vi "loadcell.vi"() -> ()   [LabVIEW 2020]
uses:
  <vilib>/DAQmx/read.llb/DAQmx Read (Analog 1D Wfm NChan NSamp).vi
  <vilib>/DAQmx/miscellaneous.llb/DAQmx Fill In Error Info.vi
panel:
  out "data 3":waveform(dbl)[](graph) caption="data"
  out "channel name(s) out":string[](array[string])
  in  "file path":path
  in  "stop":bool
  in  "data 2":waveform(dbl)[](array[waveform])
  out "data":waveform(dbl)[](graph)
  out "error out 2":errorcluster
  in  "error in (no error)":errorcluster
  out "Tare log":bool
  out "Start log":bool
  out "reconnect":bool
  out "Show message":bool
  in  "Message":string
  in  "No of Samples":dbl
  out "save Path":path
  in  "Tare":bool
  in  "Report":bool
  in  "Refresh Button":bool
  in  "Start Log":bool
  out "No of Sample":dbl
  out "Count":dbl
  out "Samples":dbl
  in  "Machine Load 3":dbl
  in  "Sample Delay":dbl
  in  "Machine Load 2":dbl
  in  "Sample Rate":dbl
  out "Part No":dbl
  out "Total Load":dbl
  out "KG 4":dbl
  out "KG 3":dbl
  out "KG 2":dbl
  out "KG":dbl
  out "Loadcell 4":bool
  out "Loadcell 3":bool
  out "Loadcell 2":bool
  out "Loadcell1":bool
  out "Loadcell 4":waveform(dbl)(graph)
  out "Loadcell 3":waveform(dbl)(graph)
  out "Loadcell 2":waveform(dbl)(graph)
  out "Loadcell1":waveform(dbl)(graph)
  # "KG"
  # "MS"
  # "Hz"
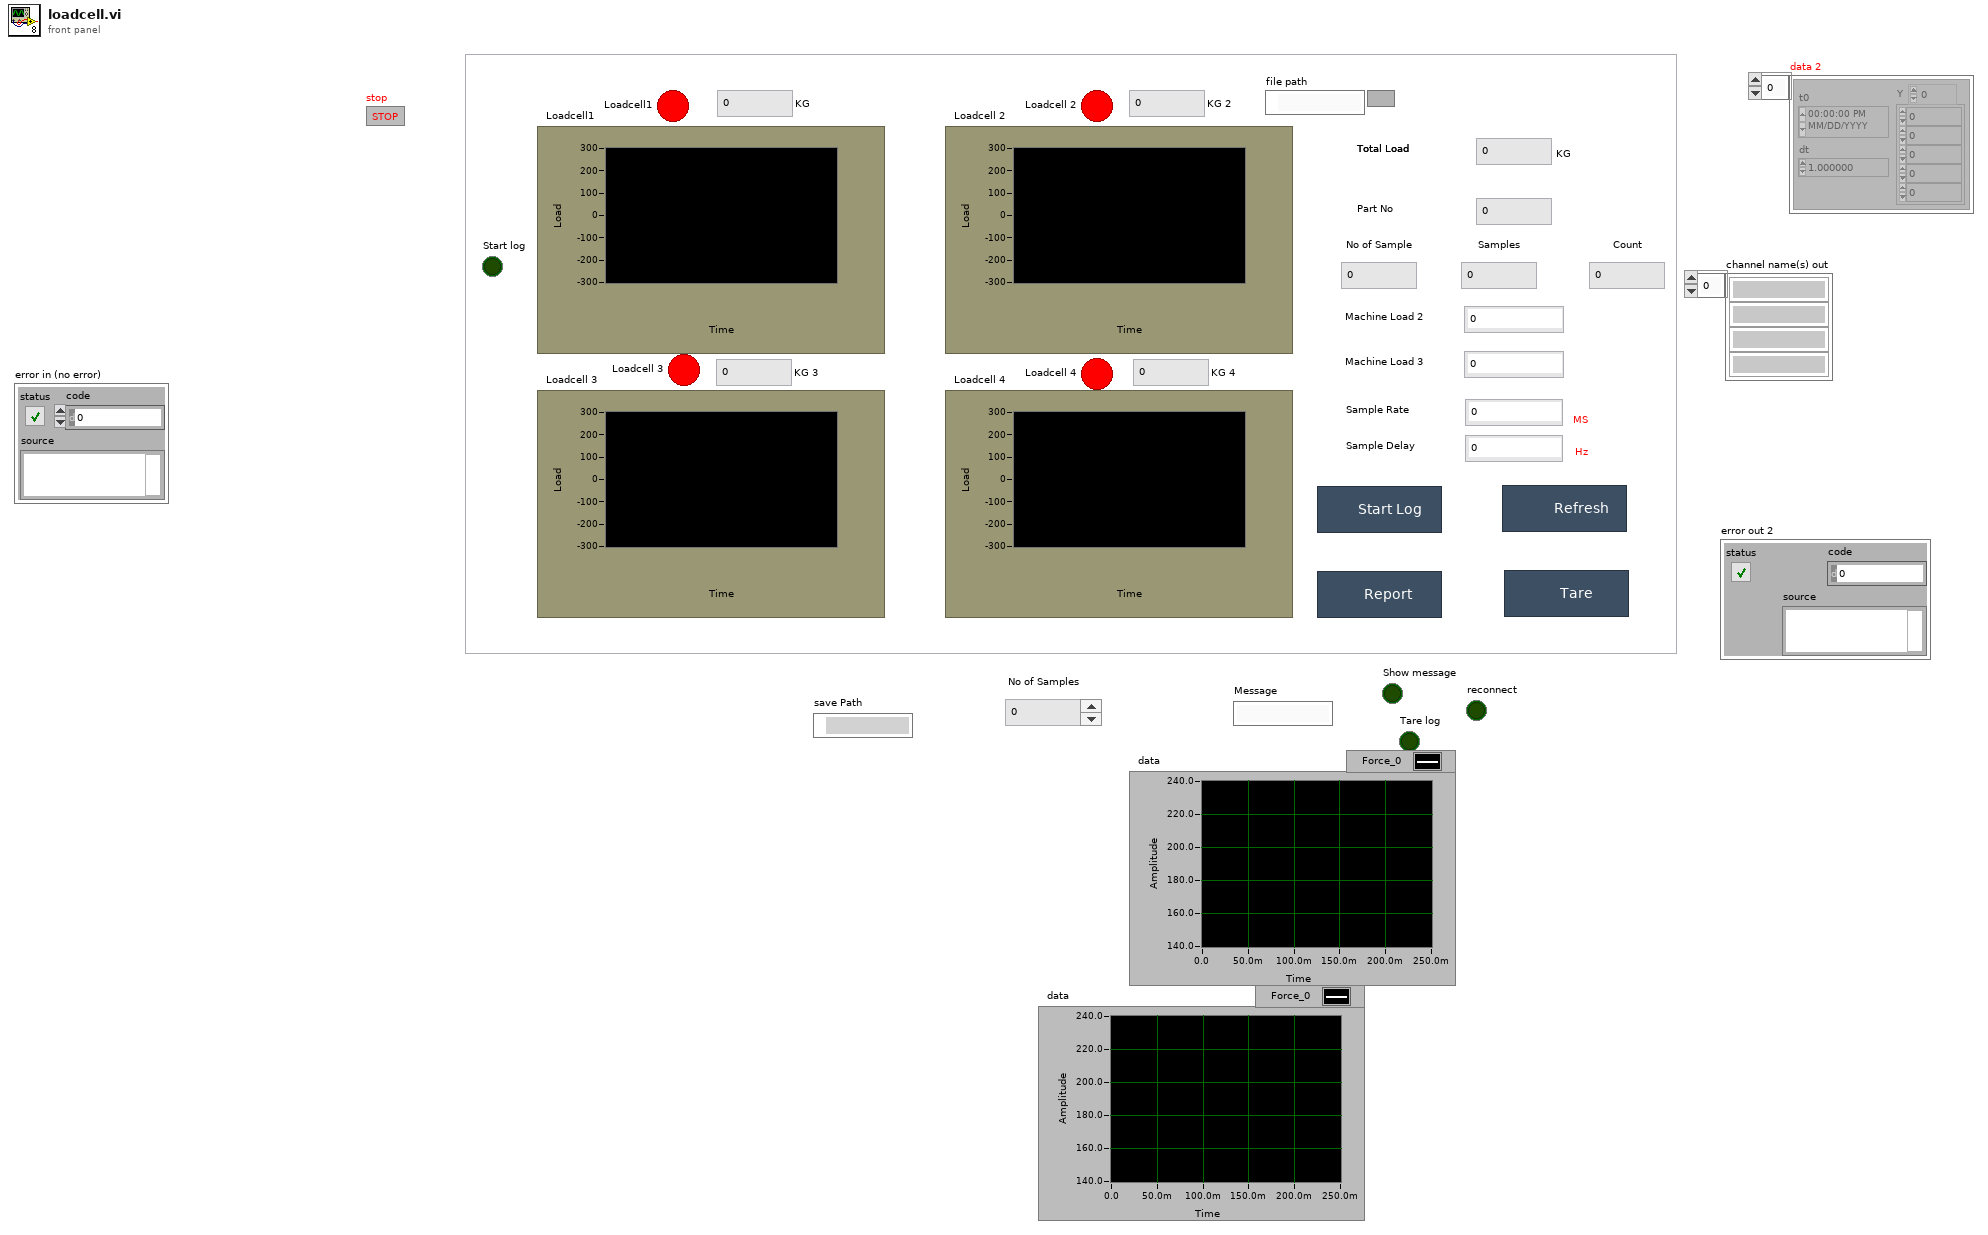
[diagram p1: front panel]
types:
  T1 = enum16{"big-endian, network order", "native, host order", "little-endian"}
  T2 = enum16{"open", "open or create", "create or replace", "create", "open (read-only)"}
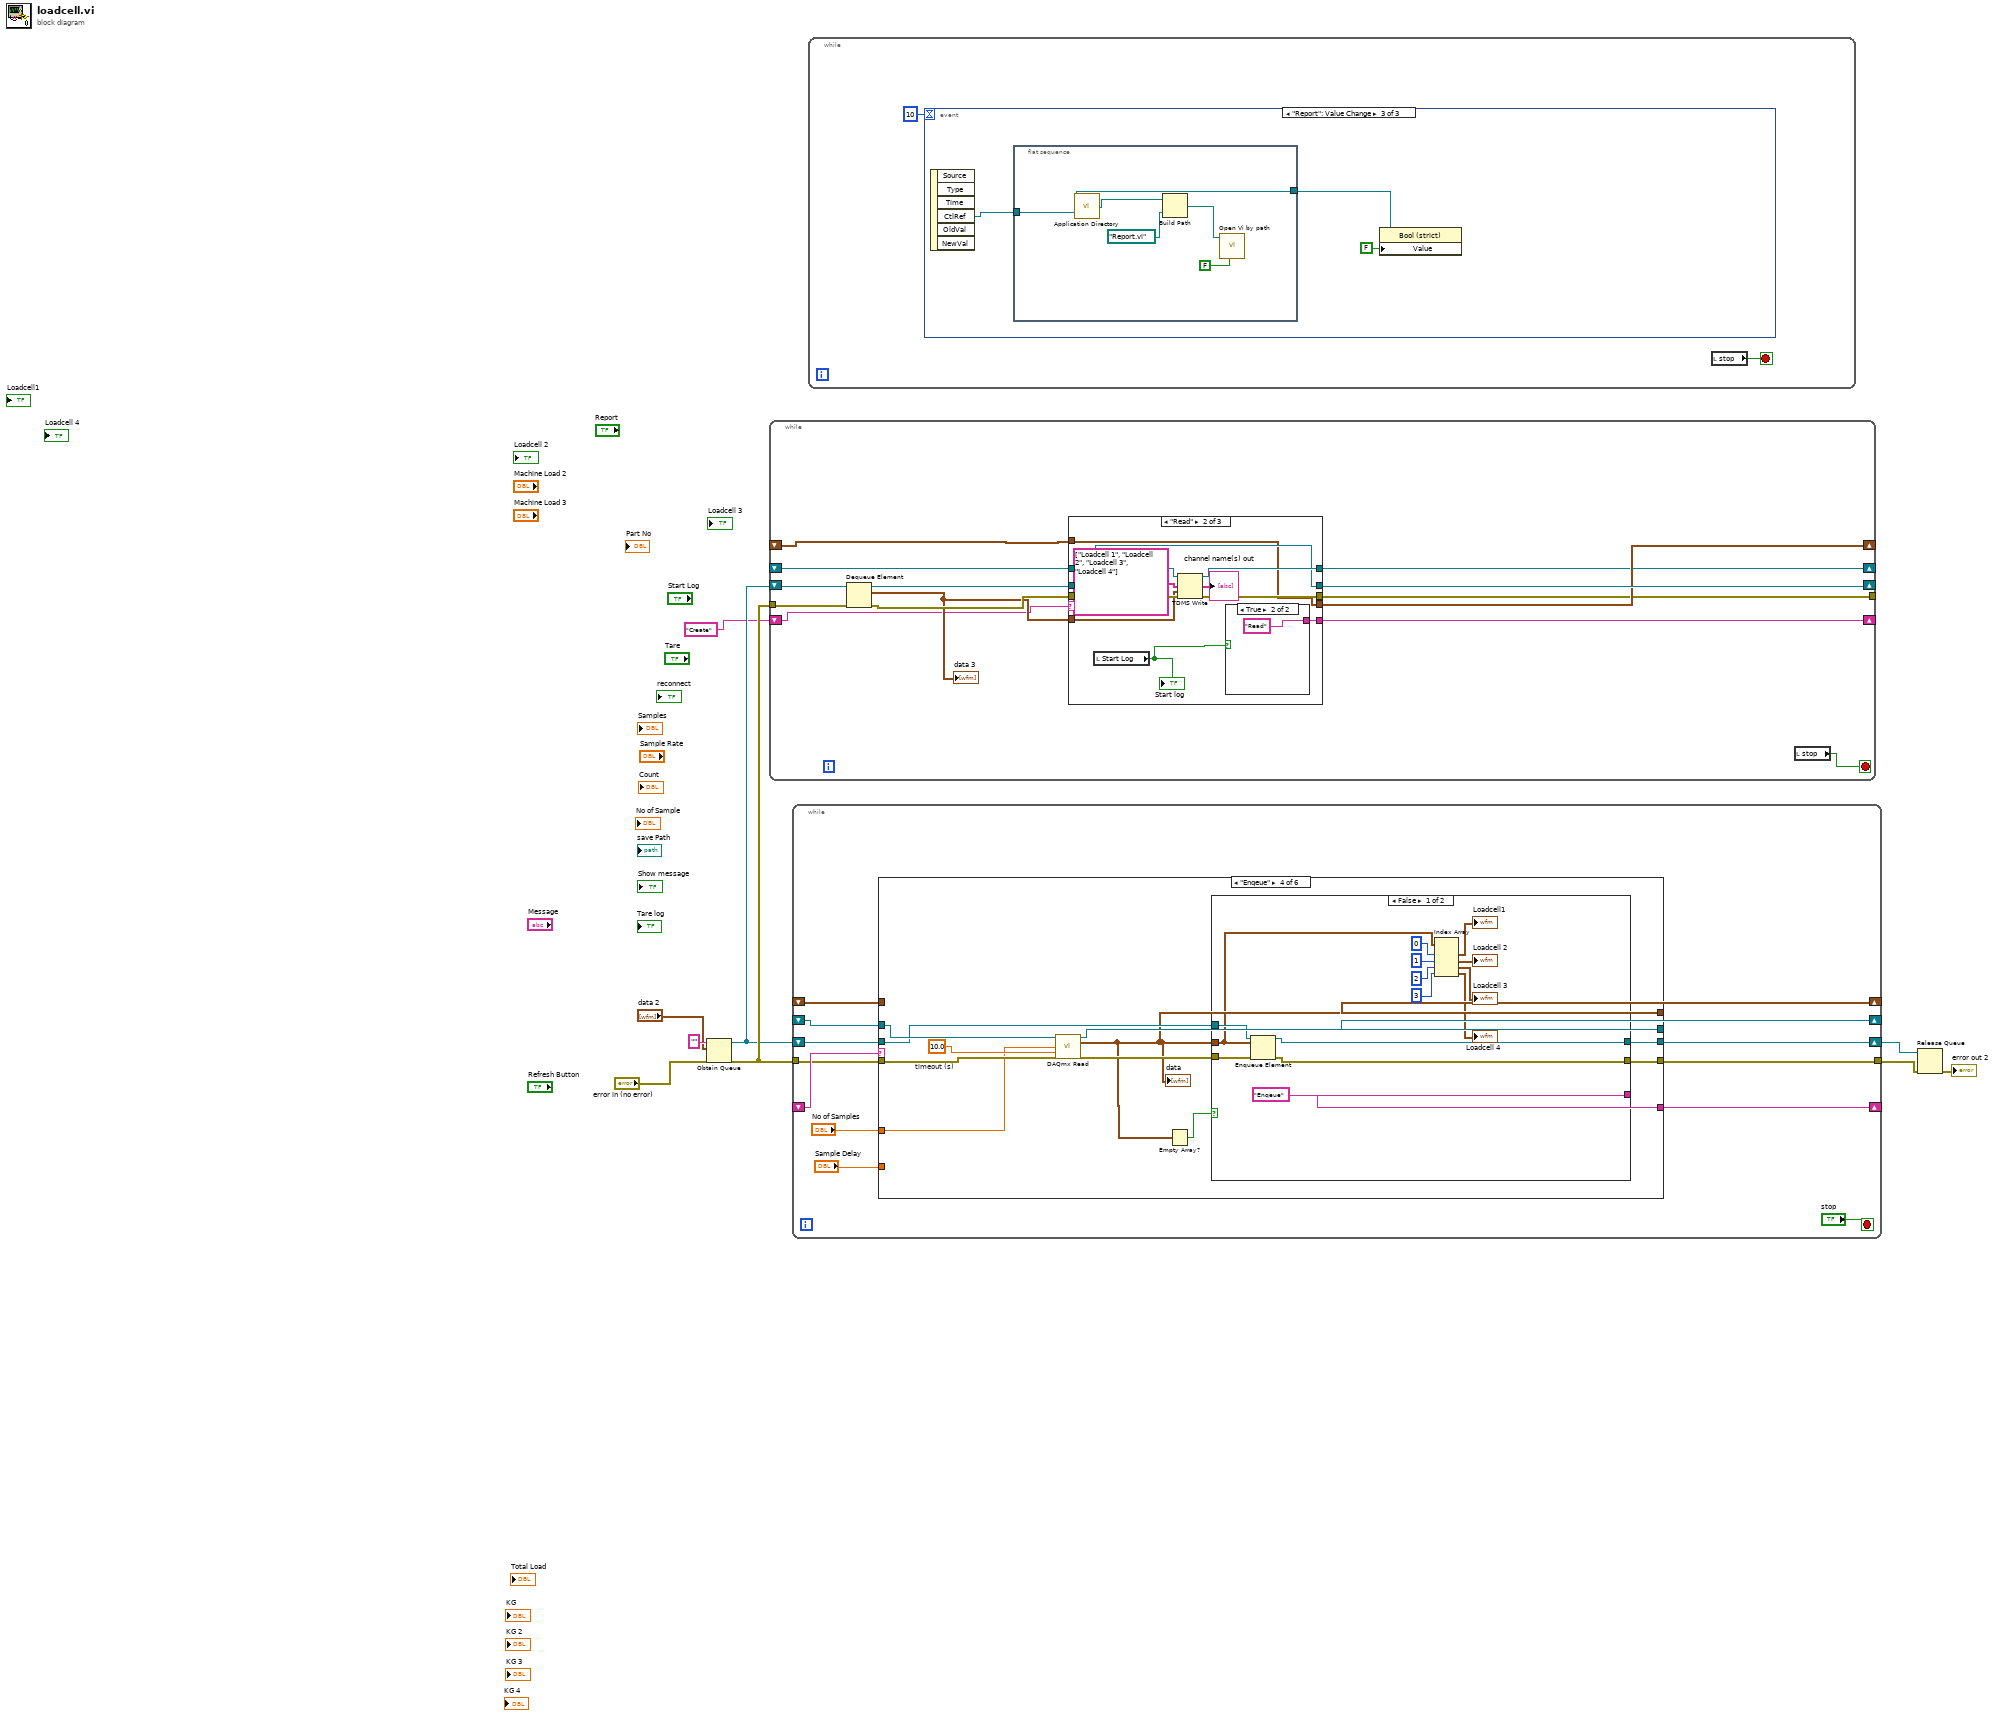
[diagram p0: block diagram]
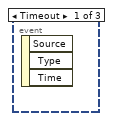
[diagram p2: hidden frame]
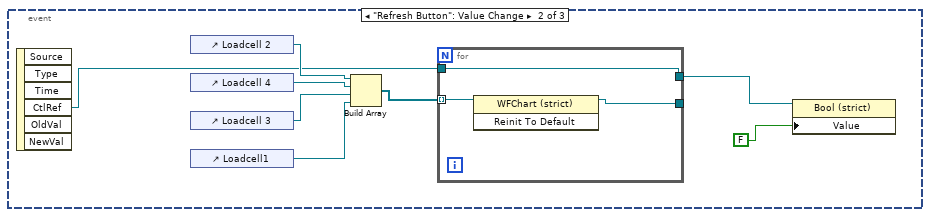
[diagram p3: hidden frame]
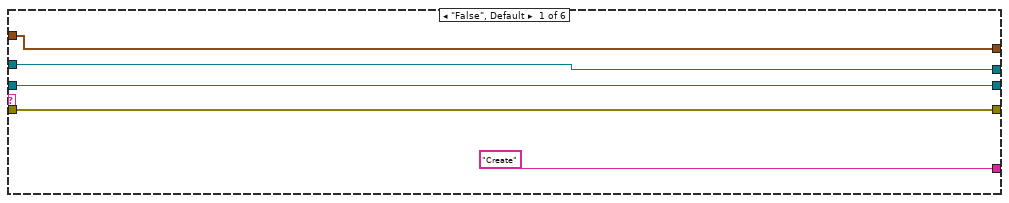
[diagram p4: hidden frame]
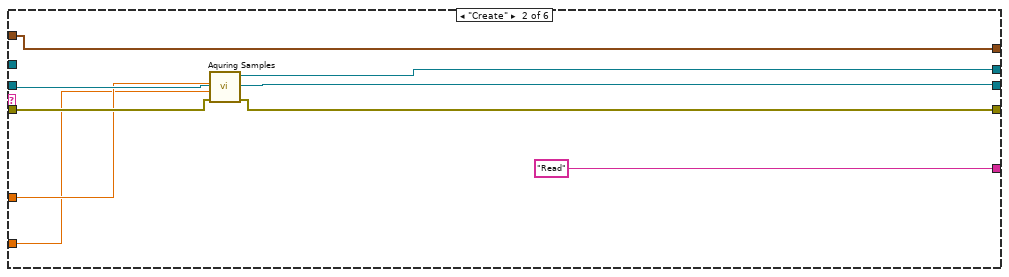
[diagram p5: hidden frame]
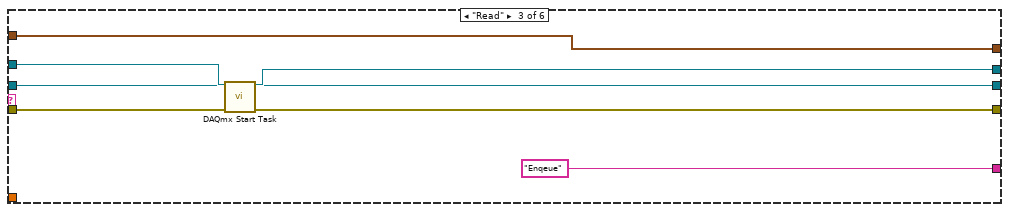
[diagram p6: hidden frame]
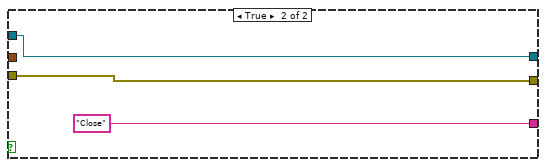
[diagram p7: hidden frame]
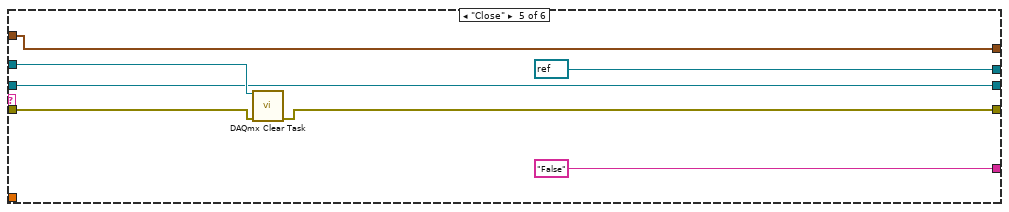
[diagram p8: hidden frame]
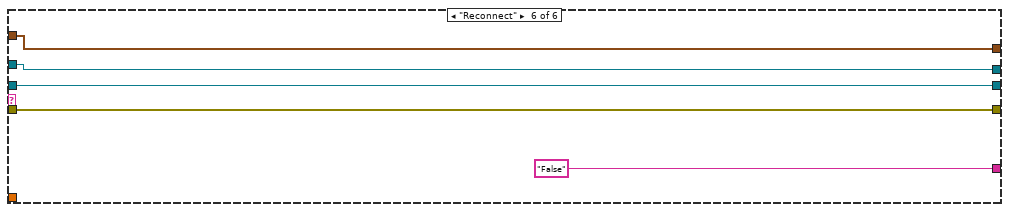
[diagram p9: hidden frame]
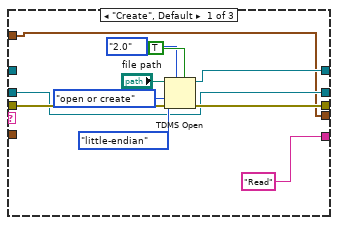
[diagram p10: hidden frame]
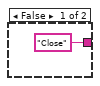
[diagram p11: hidden frame]
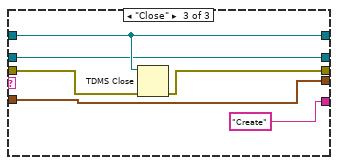
[diagram p12: hidden frame]
diagram:
  n1 = Obtain Queue(name (unnamed)="", element data type="data 2", error in (no error)="error in (no error)") -> (queue out=w2:refnum<queue>, error out=w3:errorcluster)  [unwired: 2 in, 1 out]
  n2 = while {
    tunnel: w3 -> [w22]
    shift-right: [w20] -> _
    shift-left: w2 -> [w18]
    shift-right: [w19] -> _
    shift-left: _ -> [w17]
    shift-right: [w16] -> _
    shift-left: "Create" -> [w10]
    tunnel: [w14] -> _
    shift-right: [w13] -> _
    shift-left: _ -> [w12]
    stop <- w23 stop-if-true
    n3 = Dequeue Element(queue=w18, error in (no error)=w22) -> (queue out=w21:refnum<queue>, element=w11:waveform(dbl)[], error out=w15:errorcluster)  [unwired: 1 in, 1 out]
    "data 3" <- w11
    n4 = case shown="\"Read\"" w10 {
      tunnel: ["Read" w45 "Create"] -> w16
      tunnel: w15 -> [w32 w42 w53]
      tunnel: [w27 w41 w52] -> w14
      tunnel: [w26 w43 w51] -> w13
      tunnel: w12 -> [_ w44 w51]
      tunnel: w11 -> [_ w40 w50]
      tunnel: [w24 w36 w50] -> w19
      tunnel: w21 -> [w25 w37 w49]
      tunnel: [w25 w37 w49] -> w20
      tunnel: w17 -> [w24 w36 _]
      frame "Create", Default {
        n5 = TDMS Open(5:TRUE ("create index file? (T)"), 7:enum16{"1.0", "2.0"}."2.0" ("file format version (2.0)"), 8:w32, 9:T1."little-endian" ("byte order (2:little-endian)"), 10:T2."open or create" ("operation (0:open)"), 11:"file path") -> (0:w27:errorcluster, 3:w26:refnum<k34>)  [unwired: 1 in]
      }
      frame "Read" {
        n6 = local read "Start Log"() -> (w35:bool)
        "Start log" <- w35
        n7 = TDMS Write(0:w44, 7:string[] ["Loadcell 1", "Loadcell 2", "Loadcell 3", "Loadcell 4"] ("channel name(s) in (Untitled)"), 9:w40, 11:w42) -> (4:w43:refnum<k34>, 8:→"channel name(s) out":string[], 15:w41:errorcluster)  [unwired: 2 in, 1 out]
        n8 = case shown="True" w35 {
          tunnel: ["Close" "Read"] -> w45
          frame False {
          }
          frame True {
          }
        }
      }
      frame "Close" {
        n9 = TDMS Close(8:w53, 11:w51) -> (0:w52:errorcluster)  [unwired: 1 out]
      }
    }
    n10 = local read "stop"() -> (w23:bool)
  }
  n11 = while {
    shift-right: [w63] -> _
    shift-left: _ -> [w66]
    tunnel: w3 -> [w64]
    tunnel: [w56] -> w7
    shift-right: [w55] -> w5
    shift-left: w2 -> [w65]
    shift-right: [w60] -> _
    shift-left: _ -> [w59]
    shift-right: [w57] -> _
    shift-left: _ -> [w58]
    stop <- "stop" stop-if-true
    n12 = case shown="\"Enqeue\"" w66 {
      tunnel: w65 -> [w68 w77 w82 w89 w118 w127]
      tunnel: [w68 w77 w82 w88 w118 w127] -> w55
      tunnel: w64 -> [w67 w79 w86 w96 w120 w126]
      tunnel: [w67 w78 w85 w91 w119 w126] -> w56
      tunnel: ["Create" "Read" "Enqeue" w92 "False" "False"] -> w63
      tunnel: [w69 w76 w83 w97 refnum<k21> refnum ("task out") w124] -> w60
      tunnel: "No of Samples" -> [_ w75 _ w94 _ _]
      tunnel: "Sample Delay" -> [_ w74 _ _ _ _]
      tunnel: w59 -> [w69 _ w84 w98 w121 w124]
      tunnel: [w70 w73 w80 w87 w122 w125] -> w57
      tunnel: w58 -> [w70 w73 w80 _ w122 w125]
      frame "False", Default {
      }
      frame "Create" {
        n13 = call "Aquring Samples.vi"("error in"=w79, "rate"=w74, "number of samples"=w75) -> ("error out"=w78:errorcluster, "task out"=w76:refnum<k21>)  [unwired: 7 in]
      }
      frame "Read" {
        n14 = call <vilib>:"DAQmx Start Task.vi"("task/channels in"=w84, "error in"=w86) -> ("task out"=w83:refnum<k21>, "error out"=w85:errorcluster)  [unwired: 12 in]
      }
      frame "Enqeue" {
        w95 = 10.0  # timeout (s)
        n15 = call-poly <vilib>:"DAQmx Read.vi"("task/channels in"=w98, "number of samples per channel"=w94, "timeout"=w95, "error in"=w96) -> ("task out"=w97:refnum<k21>, "data"=w87:waveform(dbl)[], "error out"=w90:errorcluster)  [unwired: 9 in]
        "data" <- w87
        n16 = Empty Array?(array=w87) -> (empty?=w93:bool)
        n17 = case shown="False" w93 {
          tunnel: ["Enqeue" "Close"] -> w92
          tunnel: w90 -> [w111 w113]
          tunnel: [w110 w113] -> w91
          tunnel: w89 -> [w109 w114]
          tunnel: [w108 w114] -> w88
          tunnel: w87 -> [w99 _]
          frame False {
            n18 = Enqueue Element(queue=w109, element=w99, error in (no error)=w111) -> (queue out=w108:refnum<queue>, error out=w110:errorcluster)  [unwired: 1 in, 1 out]
            n19 = Index Array(array=w99, index #1=0 ("index"), index #2=1 ("index"), index #3=2 ("index"), index #4=3 ("index")) -> (element #1=→"Loadcell1":waveform(dbl), element #2=→"Loadcell 2":waveform(dbl), element #3=→"Loadcell 3":waveform(dbl), element #4=→"Loadcell 4":waveform(dbl))
          }
          frame True {
          }
        }
      }
      frame "Close" {
        n20 = call <vilib>:"DAQmx Clear Task.vi"("task in"=w121, "error in"=w120) -> ("error out"=w119:errorcluster)  [unwired: 13 in]
      }
      frame "Reconnect" {
      }
    }
  }
  n21 = while {
    stop <- w128 stop-if-true
    n22 = event shown="[2] \"Report\": Value Change" {
      selector: _ -> [_ _ _]
      dyn-events: _ -> [_ _ _]
      timeout: 10 -> [_ _ _]
      event Timeout {
        n23 = event-data() -> ()  [unwired: 1 in, 3 out]
      }
      event "Refresh Button": Value Change {
        n24 = event-data() -> ("CtlRef"=w131:refnum<vi>)  [unwired: 1 in, 5 out]
        n25 = control-ref of="Loadcell 2"() -> (w136:refnum<vi>)
        n26 = control-ref of="Loadcell 4"() -> (w137:refnum<vi>)
        n27 = control-ref of="Loadcell 3"() -> (w135:refnum<vi>)
        n28 = control-ref of="Loadcell1"() -> (w134:refnum<vi>)
        n29 = Build Array(w136, w137, w135, w134) -> (w133:refnum<vi>[])
        n30 = for {
          tunnel: w133 -> [w140] mode=indexing
          tunnel: [w139] -> _
          tunnel: [w138] -> w130
          tunnel: w131 -> [w138]
          n31 = invoke class="WFChart (strict)" method="Reinit To Default"(reference=w140) -> (reference out=w139:refnum<vi>)  [unwired: 2 in, 2 out]
        }
        n32 = property class="Bool (strict)"(reference=w130, "Value"=FALSE) -> ()  [unwired: 1 in, 2 out]
      }
      event "Report": Value Change {
        n33 = event-data() -> ("CtlRef"=w143:refnum<vi>)  [unwired: 1 in, 5 out]
        n34 = flat-sequence {
          tunnel: w143 -> [w148]
          tunnel: [w148] -> w142
          frame #0 {
            n35 = call <vilib>:"Application Directory.vi"() -> ("Application Directory"=w145:path)
            n36 = Build Path(base path=w145, name or relative path=path "Report.vi") -> (appended path=w147:path)
            n37 = call "Open Vi by path.vi"("Execution:Run When Opened"=FALSE, "vi path"=w147) -> ()  [unwired: 8 in, 2 out]
          }
        }
        n38 = property class="Bool (strict)"(reference=w142, "Value"=FALSE) -> ()  [unwired: 1 in, 2 out]
      }
    }
    n39 = local read "stop"() -> (w128:bool)
  }
  n40 = Release Queue(queue=w5, error in (no error)=w7) -> (error out=→"error out 2":errorcluster)  [unwired: 1 in, 2 out]
